vi "Create Platform Application.vi"(6 "Platform Application Attributes":T1[](array[typedef]), 7 "Region":T3, 8 "error in (no error)":errorcluster, 9 "Platform":T5, 10 "Name":string, 11 "AWS Credentials":T4) -> (0 "error out":errorcluster, 3 "Platform application out":refnum<class "Platform Application.lvclass">)   [LabVIEW 2015, in "NI_AWS_SNS.lvlib" / "Platform Application.lvclass"]
doc: "Creates a platform application object for one of the supported push notification services, such as APNS and GCM, to which devices and mobile apps may register."
uses:
  Platform Application.lvclass
  Platform.ctl
  Core/HTTP Request/AWS Credentials.ctl
  Core/HTTP Request/Region.ctl
  Application Attribute Value Pair.ctl
  Application Attribute.ctl
  Core/HTTP Request/Name Value Pair.ctl
  Core/HTTP Request/Request Options.ctl
  Core/HTTP Request/Region handling.ctl
  Core/HTTP Request/URL formatting.ctl
  Core/HTTP Request/HTTP Request.lvclass
  Core/ARN/ARN.lvclass
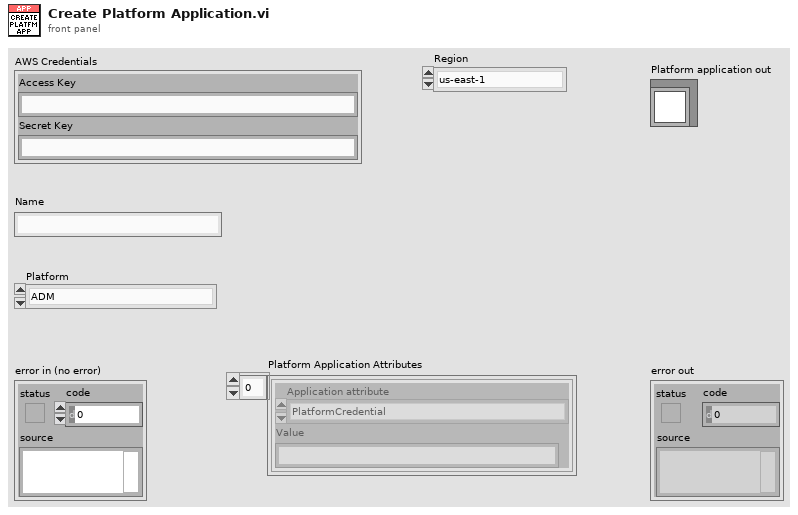
[diagram p1: front panel]
types:
  T1 = typedef "NI_AWS_SNS.lvlib/Platform Application.lvclass/Application Attribute Value Pair.ctl" = cluster{"Application attribute":T2, "Value":string}
  T2 = typedef "NI_AWS_SNS.lvlib/Platform Application.lvclass/Application Attribute.ctl" = enum16{"PlatformCredential", "PlatformPrincipal", "EventEndpointCreated", "EventEndpointDeleted", "EventEndpointUpdated", "EventDeliveryFailure", "SuccessFeedbackRoleArn", "FailureFeedbackRoleArn", "SuccessFeedbackSampleRate"}
  T3 = typedef "NI_AWS_Core.lvlib/HTTP Request.lvclass/Region.ctl" = enum16{"us-east-1", "us-east-2", "us-west-1", "us-west-2", "ap-northeast-1", "ap-northeast-2", "ap-southeast-1", "ap-southeast-2", "ca-central-1", "eu-central-1", "eu-west-1", "eu-west-2", "sa-east-1"}
  T4 = typedef "NI_AWS_Core.lvlib/HTTP Request.lvclass/AWS Credentials.ctl" = cluster{"Access Key":string, "Secret Key":string}
  T5 = typedef "NI_AWS_SNS.lvlib/Platform Application.lvclass/Platform.ctl" = enum16{"ADM", "APNS", "APNS_SANDBOX", "GCM"}
  T6 = typedef "NI_AWS_Core.lvlib/HTTP Request.lvclass/Request Options.ctl" = cluster{"request headers":T7[], "request parameters":T7[], "request body":string, "region handling":T8, "URL formatting":T9}
  T7 = typedef "NI_AWS_Core.lvlib/HTTP Request.lvclass/Name Value Pair.ctl" = cluster{"name":string, "value":string}
  T8 = typedef "NI_AWS_Core.lvlib/HTTP Request.lvclass/Region handling.ctl" = enum16{"use region everywhere", "use region (authentication only)", "use region (URL only)", "ignore region everwhere"}
  T9 = typedef "NI_AWS_Core.lvlib/HTTP Request.lvclass/URL formatting.ctl" = enum16{"region-", "region."}
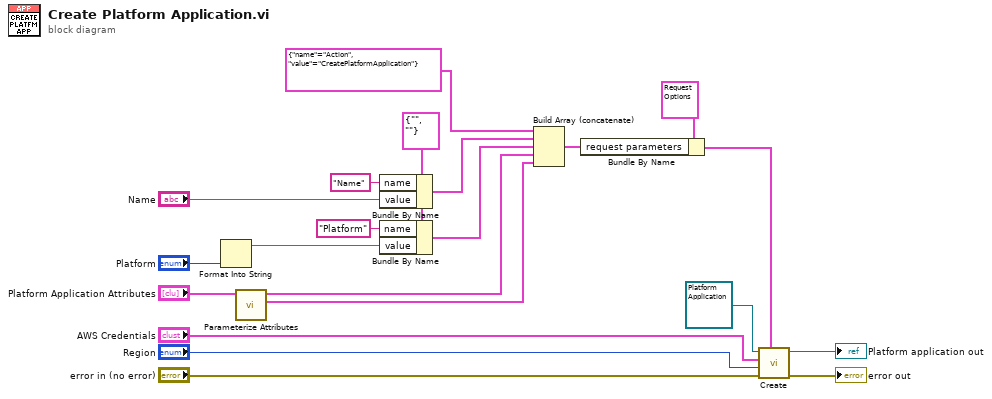
[diagram p0: block diagram]
diagram:
  w14 = T7 {"name"="", "value"=""} ("element")
  n1 = Format Into String("Platform") -> (resulting string=w11:string)  [unwired: 3 in, 1 out]
  n2 = call "Parameterize Attributes.vi"("Platform Application Attributes"="Platform Application Attributes") -> ("values"=w8:T7[], "attributes"=w9:T7[])  [unwired: 9 in]
  n3 = Bundle By Name(cluster=w14, "name"="Name", "value"="Name") -> (w15:T7)
  n4 = Bundle By Name(cluster=w14, "name"="Platform", "value"=w11) -> (w13:T7)
  n5 = Build Array (concatenate)(T7 {"name"="Action", "value"="CreatePlatformApplication"} ("Name Value Pair"), w15, w13, w9, w8) -> (w19:T7[])
  n6 = Bundle By Name(cluster=T6 {"request headers"=[], "request parameters"=[{"name"="Action", "value"="ListQueues"}], "request body"="", "region handling"=enum."use region everywhere", "URL formatting"=enum."region."} ("Request Options"), "request parameters"=w19) -> (w7:T6)
  n7 = call "Create.vi"("Request Options"=w7, "error in (no error)"="error in (no error)", "Region"="Region", "AWS Credentials"="AWS Credentials", "ARN in"=refnum<class "Platform Application.lvclass"> refnum ("NI_SNS.lvclass")) -> ("error out"=→"error out":errorcluster, "ARN out"=→"Platform application out":refnum<class "Platform Application.lvclass">)  [unwired: 5 in]
